vi "Lab 3.vi"() -> ()   [LabVIEW 2025]
uses:
  Lab 3/Control Runners.ctl
  Lab 3/Control og.ctl
  Lab 3/Control Raw.ctl
  <vilib>/Analysis/baseanly.llb/Mean (DBL).vi
  <vilib>/Analysis/NI_AALBase.lvlib
panel:
  out "error out":errorcluster
  in  "error in":errorcluster
  in  "Runner's Data":T1
  in  "File Path":path
  out "HEART RATE ZONES":string[][](array[string])
  out "BPM":cluster{"Time":timestamp[], "Bpm":i32[]}(graph)
  out "XY Graph":T2(graph)
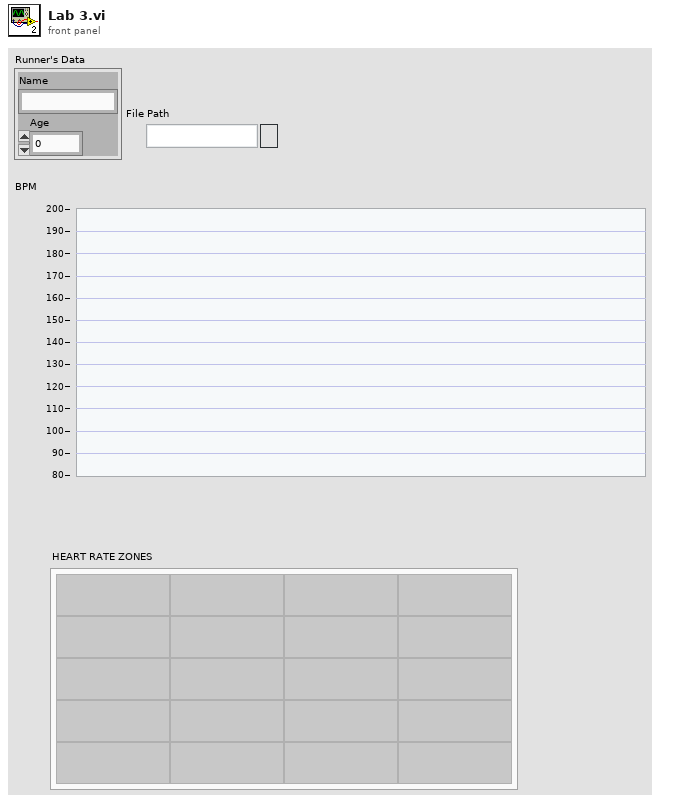
[diagram p1: front panel]
types:
  T1 = typedef "Control Runners.ctl" = cluster{"Name":string, "Age":i32}
  T2 = cluster{"Total Time in Zone":dbl[], "Heart Rate Zone No":dbl[]}
  T3 = typedef "Control og.ctl" = cluster{"Runner's Data":T1, "HR Max":i32, "Raw Data":T4, "% HR MAX ":dbl[], "HR Zones":string[][], "Heart Rate Zone No":dbl[], "Total Time in Zone":dbl[]}
  T4 = typedef "Control Raw.ctl" = cluster{"Time":timestamp[], "Bpm":i32[]}
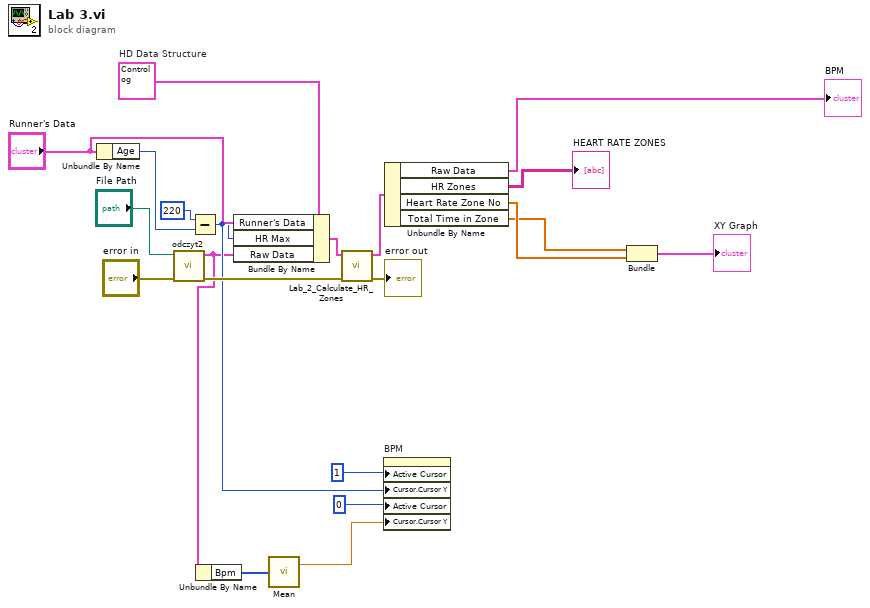
[diagram p0: block diagram]
diagram:
  w19 = T3 data[18182B]  # HD Data Structure
  n1 = Unbundle By Name("Runner's Data") -> ("Age"=w17:i32)
  n2 = call "odczyt2.vi"("error in"="error in", "Path"="File Path") -> ("error out"=w15:errorcluster, "Raw Data"=w3:T4)  [unwired: 8 in]
  n3 = Subtract(x=220, y=w17) -> (x-y=w4:i32)
  n4 = Unbundle By Name(w3) -> ("Bpm"=w2:i32[])
  n5 = Bundle By Name(cluster=w19, "Runner's Data"="Runner's Data", "HR Max"=w4, "Raw Data"=w3) -> (w13:T3)
  n6 = call-poly <vilib>:"Mean.vi"("X"=w2) -> ("mean"=w1:dbl)  [unwired: 1 out]
  n7 = call "Lab_2_Calculate_HR_Zones.vi"("error in"=w15, "HD Data Structure Control"=w13) -> ("error out"=→"error out":errorcluster, "HD Data Structure Indicator"=w12:T3)  [unwired: 8 in]
  n8 = property on="BPM" class="XYGraph (strict)"("Active Cursor"=u32 1, "Cursor.Cursor Y"=w4, "Active Cursor"=u32 0, "Cursor.Cursor Y"=w1) -> ()  [unwired: 2 in, 2 out]
  n9 = Unbundle By Name(w12) -> ("Raw Data"=→"BPM":T4, "HR Zones"=→"HEART RATE ZONES":string[][], "Heart Rate Zone No"=w9:dbl[], "Total Time in Zone"=w8:dbl[])
  n10 = Bundle("Total Time in Zone"=w8, "Heart Rate Zone No"=w9) -> (→"XY Graph":T2)  [unwired: 1 in]
